vi "Ports To System Definition.vi"(8 "error in":errorcluster, 9 "ports":T2[](array[typedef]), 10 "parameter configuration file path":path, 11 "custom device ref":T1 format="%.0x") -> (0 "error out":errorcluster, 3 "custom device ref out":T1 format="%.0x")   [LabVIEW 2020, in "Ballard ARINC 429 Scripting.lvlib"]
uses:
  Ballard ARINC 429 Scripting.lvlib
  <vilib>/NI VeriStand/Custom Device API/Custom Device Item Ref.ctl
  Shared/VS Channels Definition for All Labels on Hardware Channel.ctl
  Shared/Direction.ctl
  Shared/VS Channels Definition for Label.ctl
  Shared/VS Channel Definition for Parameter.ctl
  Shared/Parameter Definition.ctl
  <vilib>/NI/NI VeriStand Encoding and Decoding/Encoding.ctl
  Shared/Transfer Type.ctl
  Shared/Transfer Speed.ctl
  <vilib>/NI VeriStand/Custom Device API/Custom Device API.lvlib
  <vilib>/NI/VeriStand Custom Device Serialization/Custom Device Serialization.lvlib
  <vilib>/NI/NI VeriStand Encoding and Decoding/Encoding and Decoding.lvlib
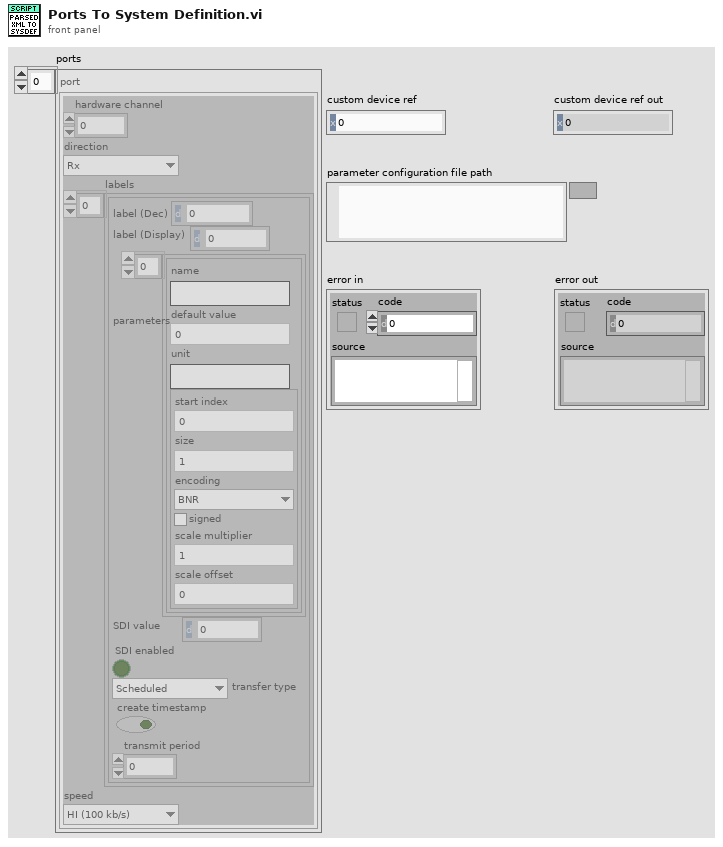
[diagram p1: front panel]
types:
  T1 = typedef "Custom Device API.lvlib/Custom Device Item Ref.ctl" = u64
  T2 = typedef "VS Channels Definition for All Labels on Hardware Channel.ctl" = cluster{"hardware channel":i32, "direction":T3, "labels":T4[], "speed":T9}
  T3 = typedef "Direction.ctl" = enum16{"Rx", "Tx"}
  T4 = typedef "VS Channels Definition for Label.ctl" = cluster{"label (Dec)":u32, "label (Display)":u32, "parameters":T5[], "SDI value":u8, "SDI enabled":bool, "transfer type":T8, "create timestamp":bool, "transmit period":u32}
  T5 = typedef "VS Channel Definition for Parameter.ctl" = cluster{"name":string, "default value":dbl, "unit":string, "Parameter":T6}
  T6 = typedef "Parameter Definition.ctl" = cluster{"start index":i32, "size":i32, "encoding":T7, "signed":bool, "scale multiplier":dbl, "scale offset":dbl}
  T7 = typedef "Encoding and Decoding.lvlib/Encoding.ctl" = enum16{"BNR", "BCD", "Discrete"}
  T8 = typedef "Transfer Type.ctl" = enum16{"Scheduled", "Acyclic", "Block", "Strobe"}
  T9 = typedef "Transfer Speed.ctl" = enum16{"LO (12.5 kb/s)", "HI (100 kb/s)"}
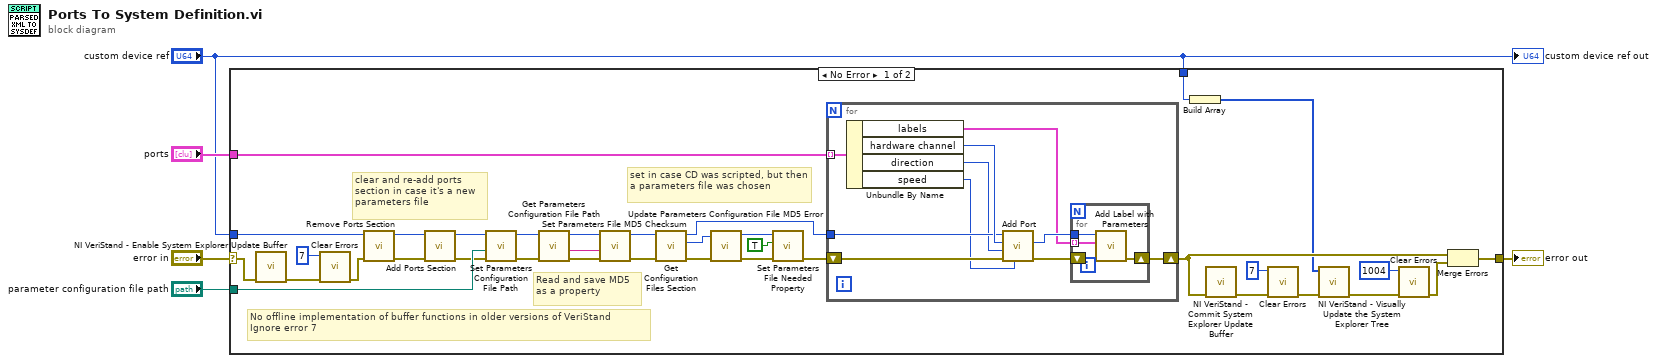
[diagram p0: block diagram]
diagram:
  n1 = case shown="No Error" "error in" {
    selector: "error in" -> [w19 w55]
    tunnel: "custom device ref" -> [w38 _]
    tunnel: [w14 w55] -> w5
    tunnel: "ports" -> [w40 _]
    tunnel: "parameter configuration file path" -> [w39 _]
    tunnel: "custom device ref" -> [w10 _]
    frame No Error {
      # "No offline implementation of buffer functions in older versions of VeriStand\nIgnore error 7"
      # "set in case CD was scripted, but then a parameters file was chosen"
      # "Read and save MD5 as a property"
      # "clear and re-add ports section in case it's a new parameters file"
      n2 = call <vilib>:"NI VeriStand - Enable System Explorer Update Buffer.vi"("error in (no error)"=w19) -> ("error out"=w18:errorcluster)  [unwired: 10 in]
      n3 = call <vilib>:"Clear Errors.vi"("error in (no error)"=w18, "specific error code to clear (0: all)"=7) -> ("error out"=w17:errorcluster)  [unwired: 4 in, 1 out]
      n4 = call "Remove Ports Section.vi"("error in"=w17, "custom device ref"=w38) -> ("error out"=w37:errorcluster, "custom device ref out"=w36:T1)  [unwired: 8 in]
      n5 = call "Add Ports Section.vi"("error in"=w37, "custom device ref"=w36) -> ("error out"=w34:errorcluster, "custom device ref out"=w35:T1)  [unwired: 7 in, 1 out]
      n6 = call "Set Parameters Configuration File Path.vi"("error in"=w34, "parameters configuration file path"=w39, "Ballard ARINC 429 custom device in"=w35) -> ("error out"=w24:errorcluster, "Ballard ARINC 429 custom device out"=w23:T1)  [unwired: 7 in]
      n7 = call "Get Parameters Configuration File Path.vi"("error in"=w24, "Ballard ARINC 429 custom device in"=w23) -> ("error out"=w32:errorcluster, "MD5 checksum"=w31:string, "Ballard ARINC 429 custom device  out"=w33:T1)  [unwired: 6 in, 1 out]
      n8 = call "Set Parameters File MD5 Checksum.vi"("error in"=w32, "MD5"=w31, "custom device ref"=w33) -> ("error out"=w29:errorcluster, "custom device ref out"=w30:T1)  [unwired: 7 in]
      n9 = call "Get Configuration Files Section.vi"("error in"=w29, "Custom device Ref"=w30) -> ("error out"=w28:errorcluster, "Configuration files Ref"=w27:T1, "Custom device Ref out"=w26:T1)  [unwired: 7 in]
      n10 = call "Update Parameters Configuration File MD5 Error.vi"("error in"=w28, "configuration files ref"=w27) -> ("error out"=w22:errorcluster, "configuration files ref out"=w20:T1)  [unwired: 8 in]
      n11 = call "Set Parameters File Needed Property.vi"("error in"=w22, "needed"=TRUE, "configuration files ref"=w20) -> ("error out"=w21:errorcluster)  [unwired: 7 in, 1 out]
      n12 = for {
        shift-right: [w47] -> w13
        shift-left: w21 -> [w44]
        tunnel: w26 -> [w45]
        tunnel: w40 -> [w50] mode=indexing
        n13 = Unbundle By Name(w50) -> ("labels"=w43:T4[], "hardware channel"=w46:i32, "direction"=w42:T3, "speed"=w41:T9)
        n14 = call "Add Port.vi"("speed (HI 100 kb/s)"=w41, "error in"=w44, "direction"=w42, "port number"=w46, "Ballard ARINC 429 custom device in"=w45) -> ("error out"=w49:errorcluster, "port"=w48:T1)  [unwired: 4 in, 1 out]
        n15 = for {
          tunnel: w48 -> [w53]
          tunnel: w43 -> [w51] mode=indexing
          shift-right: [w52] -> w47
          shift-left: w49 -> [w54]
          n16 = call "Add Label with Parameters.vi"("error in"=w54, "label"=w51, "port ref"=w53) -> ("error out"=w52:errorcluster)  [unwired: 7 in, 1 out]
        }
      }
      n17 = Build Array(w10) -> (w9:T1[])
      n18 = call <vilib>:"NI VeriStand - Commit System Explorer Update Buffer.vi"("error in (no error)"=w13) -> ("error out"=w7:errorcluster)  [unwired: 10 in]
      n19 = call <vilib>:"Clear Errors.vi"("error in (no error)"=w7, "specific error code to clear (0: all)"=7) -> ("error out"=w6:errorcluster)  [unwired: 4 in, 1 out]
      n20 = call <vilib>:"NI VeriStand - Visually Update the System Explorer Tree.vi"("error in (no error)"=w6, "Node IDs"=w9) -> ("error out"=w11:errorcluster)  [unwired: 9 in]
      n21 = call <vilib>:"Clear Errors.vi"("error in (no error)"=w11, "specific error code to clear (0: all)"=1004) -> ("error out"=w12:errorcluster)  [unwired: 4 in, 1 out]
      n22 = Merge Errors(w13, w12) -> (w14:errorcluster)
    }
    frame Error {
    }
  }
  "error out" <- w5
  "custom device ref out" <- "custom device ref"
